vi "Create LVClass Copy.vi"(5 "Override existing":bool, 6 "New Name":string, 7 "Use Relative":bool, 8 "error in (no error)":errorcluster, 9 "New Path":string, 10 "Source Class Path":path, 11 "Application in":refnum<vi>) -> (0 "error out":errorcluster, 2 "Copy Class Path out":path, 3 "Application reference out":refnum<vi>)   [LabVIEW 2019, in "gRPC Template Creation Utility.lvlib"]
uses:
  gRPC Template Creation Utility.lvlib
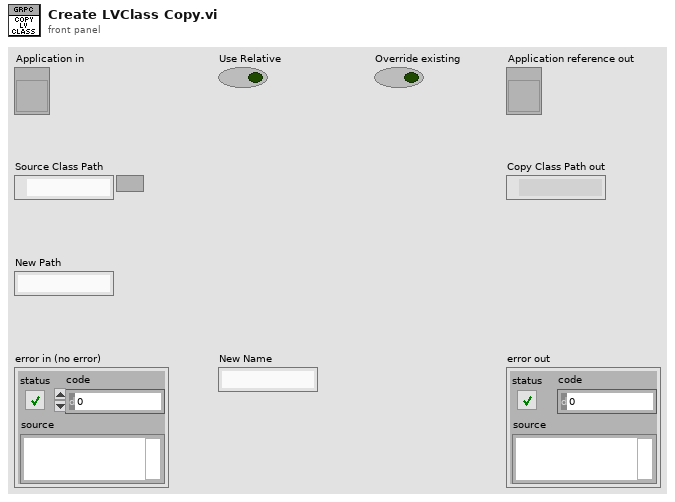
[diagram p1: front panel]
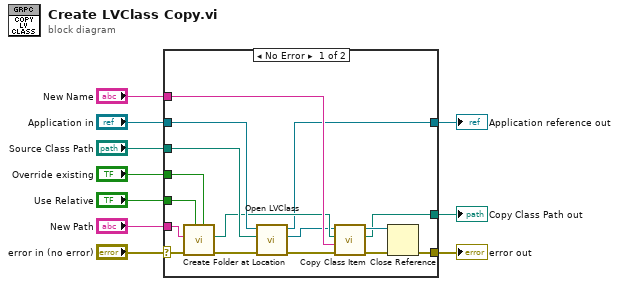
[diagram p0: block diagram]
diagram:
  n1 = case shown="No Error" "error in (no error)" {
    selector: "error in (no error)" -> [w13 w28]
    tunnel: "Use Relative" -> [w26 _]
    tunnel: "Override existing" -> [w25 _]
    tunnel: "Application in" -> [w24 w27]
    tunnel: "Source Class Path" -> [w23 _]
    tunnel: "New Name" -> [w22 _]
    tunnel: "New Path" -> [w20 _]
    tunnel: [w18 w27] -> w4
    tunnel: [w15 _] -> w3
    tunnel: [w14 w28] -> w2
    frame No Error {
      n2 = call "Create Folder at Location.vi"("Override existing (F)"=w25, "Use Relative (F)"=w26, "Error In"=w13, "Path"=w20) -> ("Error Out"=w12:errorcluster, "Full path out"=w21:path)  [unwired: 5 in, 1 out]
      n3 = call "Open LVClass.vi"("error in (no error)"=w12, "Full Path"=w23, "Application reference in"=w24) -> ("error out"=w11:errorcluster, "LVClass out"=w19:refnum<vi>, "Application reference out"=w18:refnum<vi>)  [unwired: 6 in]
      n4 = call "Copy Class Item.vi"("error in (no error)"=w11, "New Name"=w22, "Full path in"=w21, "LVClassLibrary in"=w19) -> ("error out"=w17:errorcluster, "New Class Path out"=w15:path, "LVClassLibrary out"=w16:refnum<vi>)  [unwired: 5 in]
      n5 = Close Reference(reference=w16, error in (no error)=w17) -> (error out=w14:errorcluster)
    }
    frame Error {
    }
  }
  "Copy Class Path out" <- w3
  "Application reference out" <- w4
  "error out" <- w2
